vi "AdvanceToNextProjectItem.vi"(8 "error in (no error)":errorcluster, 11 "BuildManager in":refnum<class "BuildManager.lvclass">) -> (0 "error out":errorcluster, 3 "BuildManager out":refnum<class "BuildManager.lvclass">)   [LabVIEW 2019, in "SolutionBuilder.lvlib" / "BuildManager.lvclass"]
uses:
  BuildManager.lvclass
  BuildManager.lvclass/BuildManager.ctl
  ProjectItem/ProjectItem.lvclass/ProjectItem.ctl
  ProjectItem/ProjectItem.lvclass
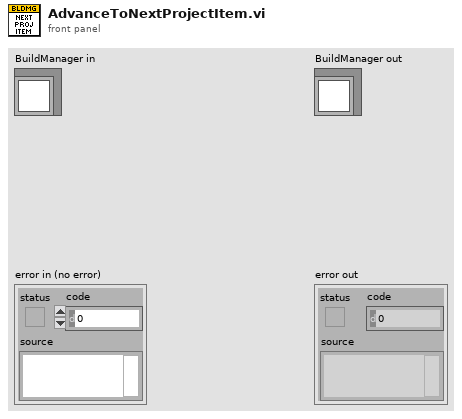
[diagram p1: front panel]
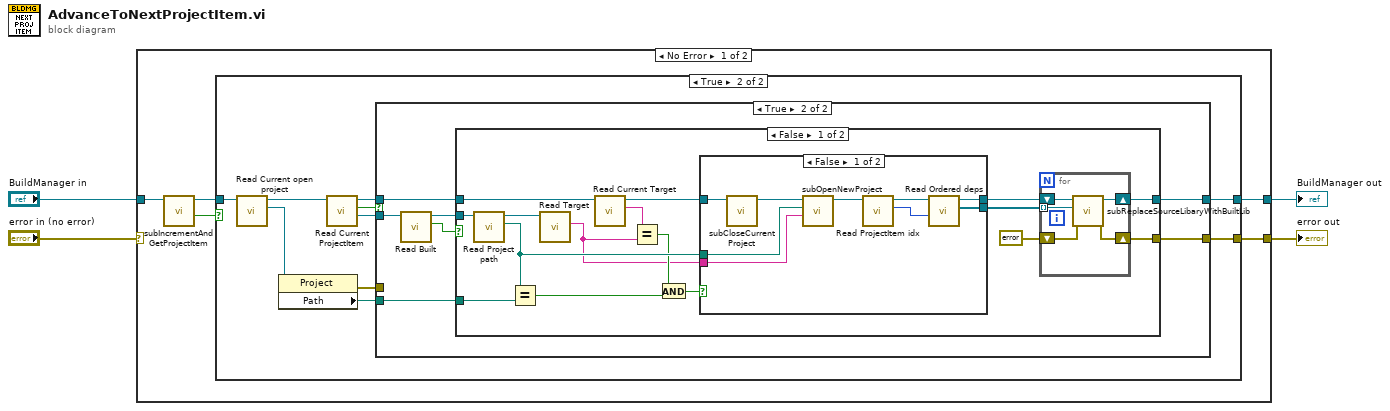
[diagram p0: block diagram]
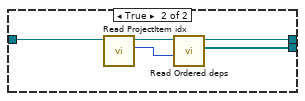
[diagram p4: hidden frame]
diagram:
  n1 = case shown="No Error" "error in (no error)" {
    selector: "error in (no error)" -> [_ w65]
    tunnel: [w9 w66] -> w4
    tunnel: "BuildManager in" -> [w8 w66]
    tunnel: [w5 w65] -> w1
    frame No Error {
      n2 = call "subIncrementAndGetProjectItem.vi"("BuildManager in"=w8) -> ("Valid"=w6:bool, "BuildManager out"=w7:refnum<class "BuildManager.lvclass">)  [unwired: 8 in, 1 out]
      n3 = case shown="True" w6 {
        tunnel: [w10 w19] -> w9
        tunnel: w7 -> [w10 w17]
        tunnel: [_ w12] -> w5
        frame False {
        }
        frame True {
          n4 = call-dynamic "Read Current open project.vi"("BuildManager in"=w17) -> ("Current open project"=w18:refnum<vi>, "BuildManager out"=w16:refnum<class "BuildManager.lvclass">)  [unwired: 9 in]
          n5 = property class="Project"(reference=w18) -> (error out=w11:errorcluster, "Path"=w20:path)  [unwired: 1 in, 1 out]
          n6 = call-dynamic "Read Current ProjectItem.vi"("BuildManager in"=w16) -> ("Current ProjectItem"=w13:refnum<class "ProjectItem.lvclass">, "Valid"=w14:bool, "BuildManager out"=w15:refnum<class "BuildManager.lvclass">)  [unwired: 7 in, 1 out]
          n7 = case shown="True" w14 {
            tunnel: w20 -> [_ w28]
            tunnel: [w21 w27] -> w19
            tunnel: w15 -> [w21 w26]
            tunnel: w13 -> [_ w24]
            tunnel: [_ w23] -> w12
            tunnel: w11 -> [_ _]
            frame False {
            }
            frame True {
              n8 = call-dynamic "Read Built.vi"("ProjectItem in"=w24) -> ("Built"=w22:bool, "ProjectItem out"=w25:refnum<class "ProjectItem.lvclass">)  [unwired: 9 in]
              n9 = case shown="False" w22 {
                tunnel: w28 -> [w44 _]
                tunnel: [w29 w64] -> w27
                tunnel: w26 -> [w37 w64]
                tunnel: w25 -> [w41 _]
                tunnel: [w39 _] -> w23
                frame False {
                  n10 = call-dynamic "Read Project path.vi"("ProjectItem in"=w41) -> ("Project path"=w43:path, "ProjectItem out"=w38:refnum<class "ProjectItem.lvclass">)  [unwired: 9 in]
                  n11 = Equal?(x=w43, y=w44) -> (x = y?=w33:bool)
                  n12 = call "Read Target.vi"("ProjectItem in"=w38) -> ("Target"=w31:string)  [unwired: 9 in, 1 out]
                  n13 = call "Read Current Target.vi"("BuildManager in"=w37) -> ("Current Target"=w35:string, "BuildManager out"=w36:refnum<class "BuildManager.lvclass">)  [unwired: 9 in]
                  n14 = Equal?(x=w35, y=w31) -> (x = y?=w34:bool)
                  n15 = And(x=w34, y=w33) -> (x .and. y?=w32:bool)
                  n16 = case shown="False" w32 {
                    tunnel: w36 -> [w53 w58]
                    tunnel: [w50 w56] -> w30
                    tunnel: w43 -> [w52 _]
                    tunnel: [w48 w55] -> w42
                    tunnel: w31 -> [w46 _]
                    frame False {
                      n17 = call "subCloseCurrentProject.vi"("BuildManager in"=w53) -> ("BuildManager out"=w45:refnum<class "BuildManager.lvclass">)  [unwired: 9 in, 1 out]
                      n18 = call "subOpenNewProject.vi"("Target"=w46, "Project path"=w52, "BuildManager in"=w45) -> ("BuildManager out"=w47:refnum<class "BuildManager.lvclass">)  [unwired: 7 in, 1 out]
                      n19 = call-dynamic "Read ProjectItem idx.vi"("BuildManager in"=w47) -> ("ProjectItem idx"=w49:i32, "BuildManager out"=w51:refnum<class "BuildManager.lvclass">)  [unwired: 9 in]
                      n20 = call-dynamic "Read Ordered deps.vi"("length (-1)"=w49, "BuildManager in"=w51) -> ("Ordered deps"=w48:refnum<class "ProjectItem.lvclass">[], "BuildManager out"=w50:refnum<class "BuildManager.lvclass">)  [unwired: 8 in]
                    }
                    frame True {
                      n21 = call-dynamic "Read ProjectItem idx.vi"("BuildManager in"=w58) -> ("ProjectItem idx"=w54:i32, "BuildManager out"=w57:refnum<class "BuildManager.lvclass">)  [unwired: 9 in]
                      n22 = call-dynamic "Read Ordered deps.vi"("length (-1)"=w54, "BuildManager in"=w57) -> ("Ordered deps"=w55:refnum<class "ProjectItem.lvclass">[], "BuildManager out"=w56:refnum<class "BuildManager.lvclass">)  [unwired: 8 in]
                    }
                  }
                  n23 = for {
                    shift-right: [w61] -> w29
                    shift-left: w30 -> [w62]
                    tunnel: w42 -> [w63] mode=indexing
                    shift-right: [w60] -> w39
                    shift-left: errorcluster {"status"=FALSE, "code"=0, "source"=""} ("error out") -> [w59]
                    n24 = call "subReplaceSourceLibaryWithBuiltLib.vi"("error in (no error)"=w59, "ProjectItem in"=w63, "BuildManager in"=w62) -> ("error out"=w60:errorcluster, "BuildManager out"=w61:refnum<class "BuildManager.lvclass">)  [unwired: 7 in]
                  }
                }
                frame True {
                }
              }
            }
          }
        }
      }
    }
    frame Error {
    }
  }
  "error out" <- w1
  "BuildManager out" <- w4
